vi "Get Path.vi"() -> (4 "libiox2_cif path":path)   [LabVIEW 2021, in "Iceoryx.lvlib"]
uses:
  Iceoryx.lvlib
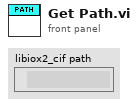
[diagram p1: front panel]
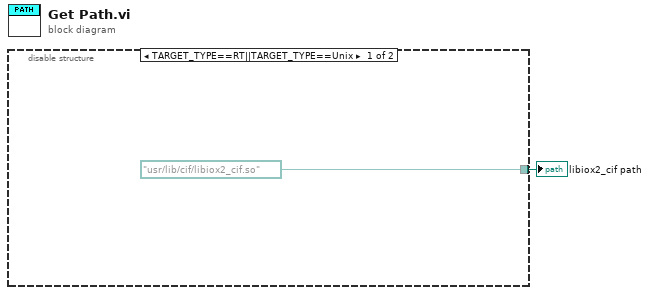
[diagram p0: block diagram]
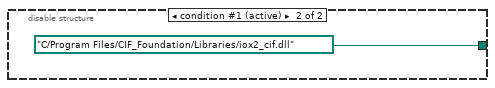
[diagram p2: hidden frame]
diagram:
  n1 = disable-structure shown="TARGET_TYPE==RT||TARGET_TYPE==Unix" {
    disable-tunnel: [path "/usr/lib/cif/libiox2_cif.so" ("file path (use dialog)") path "C:/Program Files/CIF_Foundation/Libraries/iox2_cif.dll" ("file path (use dialog)")] -> w1
    frame condition #0 {
    }
    frame condition #1 (active) {
    }
  }
  "libiox2_cif path" <- w1
